vi "RT_Servo_IO_Adapter.vi"(8 "error in (no error)":errorcluster={"status"=FALSE, "code"=0, "source"="\"\""}, 10 "hardware status":string, 11 "Motion target/mode":string) -> (0 "error out":errorcluster={"status"=FALSE, "code"=0, "source"="\"\""}, 2 "status ok":bool, 3 "Accepted/applied ACK":string)   [LabVIEW 2026]
doc: "INTENT: Implement servo amplifier communication. LOGIC: Translate target to drive units, transmit bounded command, decode statusword/encoder."
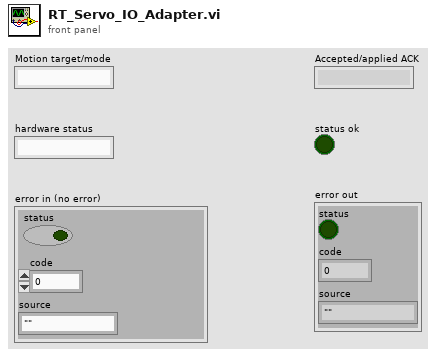
[diagram p1: front panel]
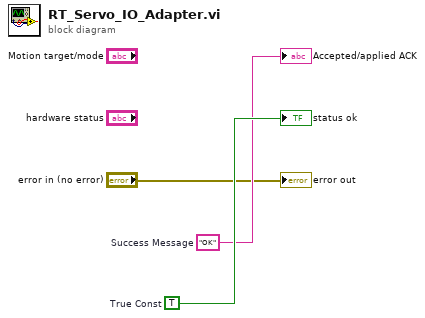
[diagram p0: block diagram]
diagram:
  w3 = TRUE  # True Const
  w2 = "OK"  # Success Message
  "Accepted/applied ACK" <- w2
  "status ok" <- w3
  "error out" <- "error in (no error)"
